vi "Media Player Example.vi"() -> ()   [LabVIEW 2017]
uses:
  Audio Player/AudioPlayer.lvclass
  ConsoleOut/Print Options.ctl
panel:
  in  "fileName":string[](array[string])=["beyond the horizon.mp3", "alone.mp4", "far far away.vlc", "mind me.avi"]
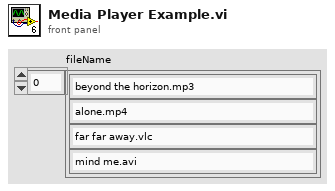
[diagram p1: front panel]
types:
  T1 = typedef "Print Options.ctl" = enum16{"Create", "Get Reference", "Print", "Print Header", "Close"}
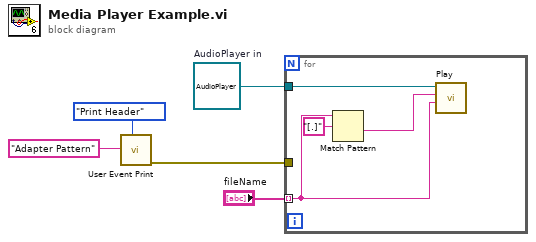
[diagram p0: block diagram]
diagram:
  w4 = refnum<class "AudioPlayer.lvclass"> refnum  # AudioPlayer in
  n1 = call "User Event Print.vi"("Options"=Print_Options."Print Header", "String to Print"="Adapter Pattern") -> ("error out"=w3:errorcluster)  [unwired: 8 in, 1 out]
  n2 = for {
    tunnel: "fileName" -> [w6] mode=indexing
    tunnel: w4 -> [w9]
    tunnel: w3 -> [_]
    n3 = Match Pattern(string=w6, regular expression="[.]") -> (after substring=w7:string)  [unwired: 1 in, 3 out]
    n4 = call-dynamic "Play.vi"("fileName"=w6, "audioType"=w7, "AudioPlayer in"=w9) -> ()  [unwired: 7 in, 2 out]
  }
